vi "VIH Utility - MENU - Recent Paths - RW INI File.vi"(4 "path delimiter (;)":string=";", 6 "cmd (read)":enum16{"read", "write"}(ring), 7 "section":string, 8 "error in":errorcluster, 9 "Menu Tags":string[](array[string]), 10 "Menu Refnum":refnum<k9>, 11 "INI refnum":T1) -> (0 "error out":errorcluster, 3 "dup INI refnum":T1)   [LabVIEW 2014]
doc: "::: VI Helpeks :::\nCopyright (c) 2000-2026 Konstantin Shifershteyn. All rights reserved."
uses:
  <vilib>/Utility/config.llb/Config Data RefNum.ctl
  <vilib>/Utility/config.llb/Write Key (String).vi
  <vilib>/Utility/config.llb/Read Key (String).vi
  <vilib>/Utility/config.llb/NI_LVConfig.lvlib
panel:
  # "VI Helpeks\nCopyright (c) 2012-2026 Konstantin Shifershteyn"
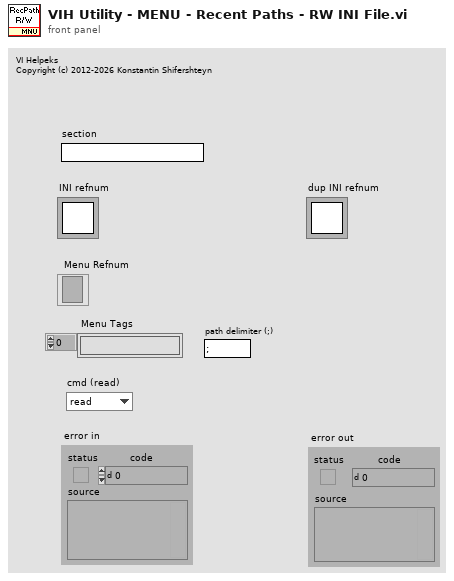
[diagram p1: front panel]
types:
  T1 = typedef "NI_LVConfig.lvlib/Config Data RefNum.ctl" = refnum<k1>
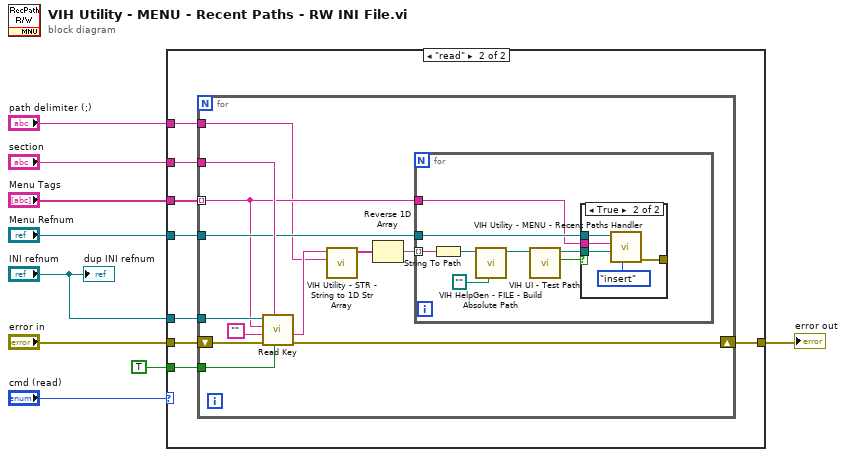
[diagram p0: block diagram]
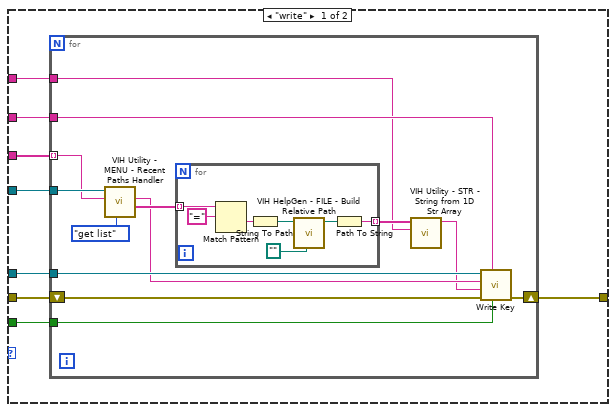
[diagram p2: hidden frame]
diagram:
  n1 = case shown="\"read\"" "cmd (read)" {
    tunnel: "section" -> [w17 w45]
    tunnel: "error in" -> [w13 w43]
    tunnel: [w14 w42] -> w3
    tunnel: "INI refnum" -> [w16 w40]
    tunnel: "Menu Refnum" -> [w15 w44]
    tunnel: "Menu Tags" -> [w12 w41]
    tunnel: "path delimiter (;)" -> [w11 w39]
    tunnel: TRUE ("read raw string? (F)") -> [w10 w38]
    frame "write" {
      n2 = for {
        tunnel: w17 -> [w30]
        tunnel: w15 -> [w25]
        shift-right: [w28] -> w14
        shift-left: w13 -> [w18]
        tunnel: w12 -> [w23] mode=indexing
        tunnel: w11 -> [w21]
        tunnel: w16 -> [w29]
        tunnel: w10 -> [w19]
        n3 = call "VIH Utility - MENU - Recent Paths Handler.vi"("cmd (get list)"=enum32{"get list", "delete", "insert"}."get list" ("cmd"), "menu tag"=w23, "menubar"=w25) -> ("item tags"=w27:string[], "dup menu tag"=w26:string)  [unwired: 5 in, 2 out]
        n4 = for {
          tunnel: w27 -> [w37] mode=indexing
          tunnel: [w32] -> w22 mode=indexing
          n5 = Match Pattern(string=w37, regular expression="=") -> (after substring=w36:string)  [unwired: 4 out]
          n6 = String To Path(string=w36) -> (path=w34:path)
          n7 = call "VIH HelpGen - FILE - Build Relative Path.vi"("Root Path"=path "", "Path in"=w34) -> ("Path out"=w33:path)  [unwired: 9 in]
          n8 = Path To String(path=w33) -> (string=w32:string)
        }
        n9 = call "VIH Utility - STR - String from 1D Str Array.vi"("delimiter ('\\n')"=w21, "Array in"=w22) -> ("String out"=w20:string)  [unwired: 5 in]
        n10 = call-poly <vilib>:"Write Key.vi"("write raw string? (F)"=w19, "section"=w30, "error in (no error)"=w18, "value"=w20, "key"=w26, "refnum"=w29) -> ("error out"=w28:errorcluster)  [unwired: 5 out]
      }
    }
    frame "read" {
      n11 = for {
        tunnel: w45 -> [w57]
        tunnel: w40 -> [w56]
        tunnel: w44 -> [w52]
        shift-right: [w46] -> w42
        shift-left: w43 -> [w50]
        tunnel: w41 -> [w49] mode=indexing
        tunnel: w39 -> [w48]
        tunnel: w38 -> [w47]
        n12 = call-poly <vilib>:"Read Key.vi"("read raw string? (F)"=w47, "section"=w57, "error in (no error)"=w50, "default value"="", "key"=w49, "refnum"=w56) -> ("error out"=w46:errorcluster, "value"=w54:string)  [unwired: 4 out]
        n13 = call "VIH Utility - STR - String to 1D Str Array.vi"("delimiter ('\\n')"=w48, "String in"=w54) -> ("Array out"=w53:string[])  [unwired: 5 in]
        n14 = Reverse 1D Array(array=w53) -> (reversed array=w51:string[])
        n15 = for {
          tunnel: w51 -> [w64] mode=indexing
          tunnel: w52 -> [w65]
          tunnel: w49 -> [w63]
          n16 = String To Path(string=w64) -> (path=w60:path)
          n17 = call "VIH HelpGen - FILE - Build Absolute Path.vi"("Root Path"=path "", "Path in"=w60) -> ("Path out"=w59:path)  [unwired: 9 in]
          n18 = call "VIH UI - Test Path.vi"("Path"=w59) -> ("Good Path"=w61:bool, "dup Path"=w62:path)  [unwired: 7 in, 2 out]
          n19 = case shown="True" w61 {
            tunnel: w65 -> [_ w70]
            tunnel: w63 -> [_ w69]
            tunnel: w62 -> [_ w68]
            tunnel: [_ w66] -> _
            frame False {
            }
            frame True {
              n20 = call "VIH Utility - MENU - Recent Paths Handler.vi"("cmd (get list)"=enum32{"get list", "delete", "insert"}."insert" ("cmd"), "Path"=w68, "menu tag"=w69, "menubar"=w70) -> ("error out"=w66:errorcluster)  [unwired: 4 in, 3 out]
            }
          }
        }
      }
    }
  }
  "error out" <- w3
  "dup INI refnum" <- "INI refnum"
